vi "[ex ce] Levenberg Marquardt fitting.vi"() -> ()   [LabVIEW 2021]
doc: "CE-Math example.\n\n::: CalcExpress Toolkit :::\nCopyright (c) 2000-2026 Konstantin Shifershteyn. All rights reserved."
uses:
  ce exmpl - 1D difference info.ctl
  <vilib>/gmath/NumericalOptimization/Nonlinear Curve Fit LM formula string.vi
  <vilib>/Analysis/NI_AALBase.lvlib
  <vilib>/gmath/NI_Gmath.lvlib
panel:
  out "GM state":string
  out "CE state":string
  out "Coef. Difference":dbl[](array[numeric]) format="%.6g"
  out "max relative difference":T1={"index"=-1, "absolute difference"=0.0, "relative difference, %"=0.0} {"relative difference, %" format="%#.6g"; "absolute difference" format="%#.6g"}
  out "max absolute difference":T1={"index"=-1, "absolute difference"=0.0, "relative difference, %"=0.0} {"relative difference, %" format="%#.6g"; "absolute difference" format="%#.6g"}
  in  "formula info":cluster{"formula":string, "x-variable":string}={"formula"="2+4*cos(x*sin(x)) + 0.7*x*x", "x-variable"="x"}
  out "speed ratio":dbl format="%.2f"
  out "Coefficients [GM]":dbl[](array[numeric]) format="%.6g"
  out "GM time, ms":u32
  out "GM graph":cluster{"X Values":dbl[], dbl[]}[](graph) caption="G Math"
  in  "noise level":dbl=5.0 format="%.2f"
  out "Coefficients [CE]":dbl[](array[numeric]) format="%#.6g"
  out "CE time, ms":u32
  in  "end":dbl=14.0 format="%.2f"
  in  "start":dbl format="%.2f"
  in  "# points":u32=1000
  in  "model description":T2={"model"="a+b*cos(x*sin(x))+c*x*x", "Parameters"=["a", "b", "c"], "x"="x"}
  out "CE graph":cluster{"X Values":dbl[], dbl[]}[](graph) caption="CalcExpress"
  in  "Initial Guess Coef.":dbl[](array[numeric])=[0.0, 0.0, 0.0] format="%.2f"
  # "NOTE    CalcExpress uses (^) operator to perform bitwise-XOR operation but not exponentiation operation.\n You have to use double-asterisk (**) operator to compute an exponent in a CalcExpress expression. For sample, x**y ."
  # "Generation parameters"
  # "Fitting model description"
  # "Coefficients computed by CalcExpress and G-Math"
  # "Max difference of Best Fit arrays"
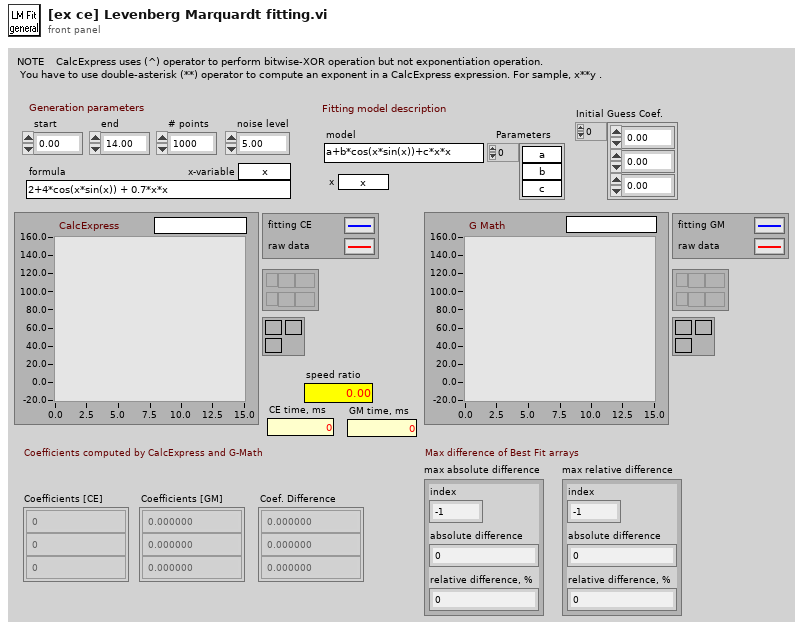
[diagram p1: front panel]
types:
  T1 = typedef "ce exmpl - 1D difference info.ctl" = cluster{"index":i32, "absolute difference":dbl, "relative difference, %":dbl}
  T2 = cluster{"model":string, "Parameters":string[], "x":string}
  T3 = cluster{"X Values":dbl[], "best nonlinear fit":dbl[]}
  T4 = cluster{"X Values":dbl[], "best nonlinear fit":dbl[]}[]
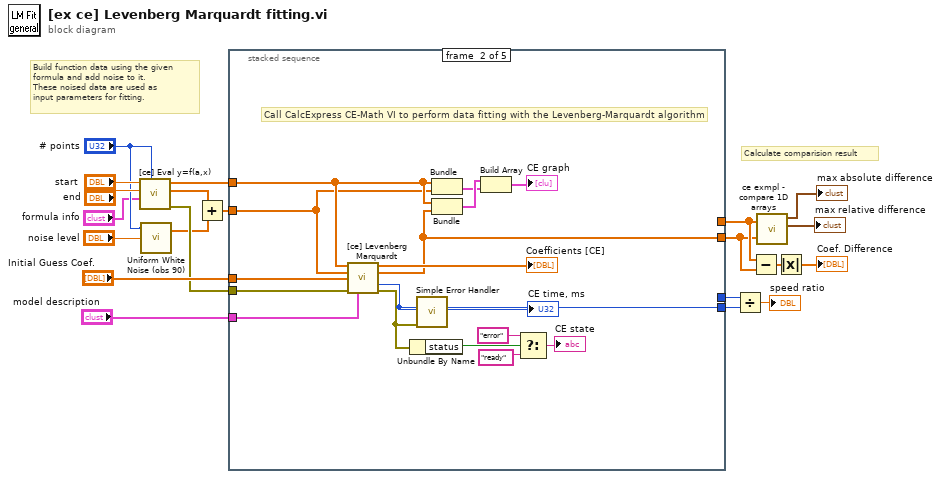
[diagram p0: block diagram]
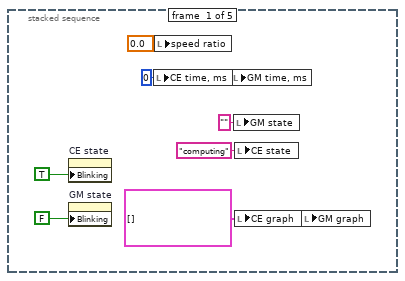
[diagram p2: hidden frame]
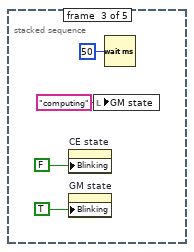
[diagram p3: hidden frame]
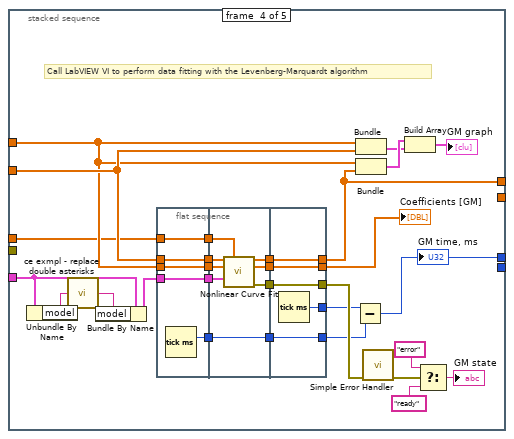
[diagram p4: hidden frame]
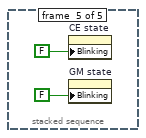
[diagram p5: hidden frame]
diagram:
  # "Calculate comparision result"
  # "Build function data using the given\nformula and add noise to it.\nThese noised data are used as\ninput parameters for fitting."
  n1 = call "[ce] Eval y=f(a,x).vi"("# points"="# points", "formula info"="formula info", "end"="end", "start"="start") -> ("error out"=w17:errorcluster, "Y Values"=w13:dbl[], "X Values"=w16:dbl[])  [unwired: 4 in, 1 out]
  n2 = call <vilib>:"Uniform White Noise (obs 90).vi"("amplitude"="noise level", "samples"="# points") -> ("uniform white noise"=w11:dbl[])  [unwired: 1 in, 1 out]
  n3 = Add(x=w13, y=w11) -> (x+y=w15:dbl[])
  n4 = stacked-sequence {
    tunnel: "Initial Guess Coef." -> [_ w44 _ w65 _]
    tunnel: "model description" -> [_ w41 _ w69 _]
    tunnel: w17 -> [_ w40 _ _ _]
    tunnel: w16 -> [_ w39 _ w67 _]
    tunnel: w15 -> [_ w38 _ w68 _]
    tunnel: [_ _ _ w49 _] -> w10
    tunnel: [_ w35 _ _ _] -> w9
    tunnel: [_ _ _ w64 _] -> w3
    tunnel: [_ w34 _ _ _] -> w2
    frame #0 {
      w24 = cluster{"X Values":dbl[], dbl[]}[] [] ("CE graph")
      w27 = u32 0 ("CE time, ms")
      n5 = property on="CE state" class="Str"("Blinking"=TRUE ("Write Attribute")) -> ()  [unwired: 2 in, 2 out]
      n6 = property on="GM state" class="Str"("Blinking"=FALSE ("Write Attribute")) -> ()  [unwired: 2 in, 2 out]
      n7 = local write "CE time, ms"(w27) -> ()
      n8 = local write "speed ratio"(0.0 ("speed ratio")) -> ()
      n9 = local write "GM time, ms"(w27) -> ()
      n10 = local write "GM state"("" ("GM state")) -> ()
      n11 = local write "CE state"("computing" ("CE state")) -> ()
      n12 = local write "CE graph"(w24) -> ()
      n13 = local write "GM graph"(w24) -> ()
    }
    frame #1 {
      # "Call CalcExpress CE-Math VI to perform data fitting with the Levenberg-Marquardt algorithm"
      n14 = call "[ce] Levenberg Marquardt.vi"("X"=w39, "Y"=w38, "Initial Guess Coefficients"=w44, "error in"=w40, "model description"=w41) -> ("Best Fit Coefficients"=→"Coefficients [CE]":dbl[], "Best Fit"=w34:dbl[], "ticks"=w35:u32, "error out"=w29:errorcluster)  [unwired: 4 in, 3 out]
      "CE time, ms" <- w35
      n15 = Unbundle By Name(w29) -> ("status"=w30:bool)
      n16 = call <vilib>:"Simple Error Handler.vi"("error in (no error)"=w29) -> ()  [unwired: 4 in, 5 out]
      n17 = Bundle("X Values"=w39, w38) -> (w36:cluster{"X Values":dbl[], dbl[]})  [unwired: 1 in]
      n18 = Bundle("X Values"=w39, "Best Fit"=w34) -> (w37:cluster{"X Values":dbl[], "Best Fit":dbl[]})  [unwired: 1 in]
      n19 = Build Array(w37, w36) -> (→"CE graph":cluster{"X Values":dbl[], "Best Fit":dbl[]}[])
      n20 = Select(t="error", s=w30, f="ready") -> (s? t:f=→"CE state":string)
    }
    frame #2 {
      n21 = property on="CE state" class="Str"("Blinking"=FALSE ("Write Attribute")) -> ()  [unwired: 2 in, 2 out]
      n22 = property on="GM state" class="Str"("Blinking"=TRUE ("Write Attribute")) -> ()  [unwired: 2 in, 2 out]
      n23 = local write "GM state"("computing" ("CE state")) -> ()
      n24 = Wait (ms)(milliseconds to wait=u32 50) -> ()  [unwired: 1 out]
    }
    frame #3 {
      # "Call LabVIEW VI to perform data fitting with the Levenberg-Marquardt algorithm"
      n25 = Unbundle By Name(w69) -> ("model"=w71:string)
      n26 = call "ce exmpl - replace double asterisks .vi"("formula in"=w71) -> ("formula out"=w70:string)  [unwired: 4 in]
      n27 = Bundle By Name(cluster=w69, "model"=w70) -> (w66:T2)
      n28 = flat-sequence {
        tunnel: w65 -> [w79]
        tunnel: w66 -> [w80]
        tunnel: w67 -> [w81]
        tunnel: w68 -> [w82]
        tunnel: [w82] -> w60
        tunnel: [w81] -> w59
        tunnel: [w80] -> w58
        tunnel: [w79] -> w57
        tunnel: [w78] -> w52
        tunnel: w60 -> [w90]
        tunnel: w59 -> [w89]
        tunnel: w58 -> [w88]
        tunnel: w57 -> [w87]
        tunnel: [w86] -> w56
        tunnel: [w85] -> w55
        tunnel: [w84] -> w54
        tunnel: w52 -> [w83]
        tunnel: [w83] -> w51
        tunnel: [w93] -> w62
        tunnel: [w94] -> w63
        tunnel: [w95] -> w64
        tunnel: w56 -> [w95]
        tunnel: w55 -> [w94]
        tunnel: w54 -> [w93]
        tunnel: [w92] -> w53
        tunnel: w51 -> [w91]
        tunnel: [w91] -> w50
        frame #0 {
          n29 = Tick Count (ms)() -> (millisecond timer value=w78:u32)
        }
        frame #1 {
          n30 = call-poly <vilib>:"Nonlinear Curve Fit.vi"("Y"=w90, "initial parameters"=w87, "X"=w89, "model description"=w88) -> ("best nonlinear fit"=w86:dbl[], "best fit parameters"=w85:dbl[], "error out"=w84:errorcluster)  [unwired: 7 in, 2 out]
        }
        frame #2 {
          n31 = Tick Count (ms)() -> (millisecond timer value=w92:u32)
        }
      }
      n32 = Subtract(x=w53, y=w50) -> (x-y=w49:u32)
      "GM time, ms" <- w49
      n33 = Bundle("X Values"=w67, w68) -> (w76:cluster{"X Values":dbl[], dbl[]})  [unwired: 1 in]
      n34 = Bundle("X Values"=w67, "best nonlinear fit"=w64) -> (w77:T3)  [unwired: 1 in]
      n35 = call <vilib>:"Simple Error Handler.vi"("error in (no error)"=w62) -> ("error out"=w61:errorcluster)  [unwired: 4 in, 4 out]
      n36 = Build Array(w77, w76) -> (→"GM graph":T4)
      n37 = Select(t="error", s=w61, f="ready") -> (s? t:f=→"GM state":string)
      "Coefficients [GM]" <- w63
    }
    frame #4 {
      n38 = property on="CE state" class="Str"("Blinking"=FALSE ("Write Attribute")) -> ()  [unwired: 2 in, 2 out]
      n39 = property on="GM state" class="Str"("Blinking"=FALSE ("Write Attribute")) -> ()  [unwired: 2 in, 2 out]
    }
  }
  n40 = Divide(x=w10, y=w9) -> (x/y=→"speed ratio":dbl)
  n41 = Subtract(x=w3, y=w2) -> (x-y=w4:dbl[])
  n42 = call "ce exmpl - compare 1D arrays.vi"("checking array B"=w2, "standard array A"=w3) -> ("max relative difference"=→"max relative difference":T1, "max absolute difference"=→"max absolute difference":T1)  [unwired: 1 in, 2 out]
  n43 = Absolute Value(x=w4) -> (abs(x)=→"Coef. Difference":dbl[])
